vi "Replace Message Specifier.vi"(11 "format string":string) -> (3 "resulting string":string)   [LabVIEW 2018, in "GLog.lvlib" / "Format String.lvclass"]
uses:
  Format String.lvclass
  <vilib>/regexp/Match Regular Expression.xnode
panel:
  # "Connector Pane"
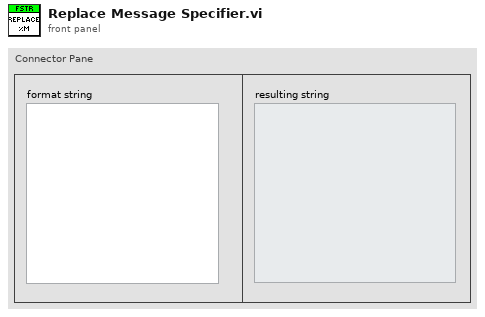
[diagram p1: front panel]
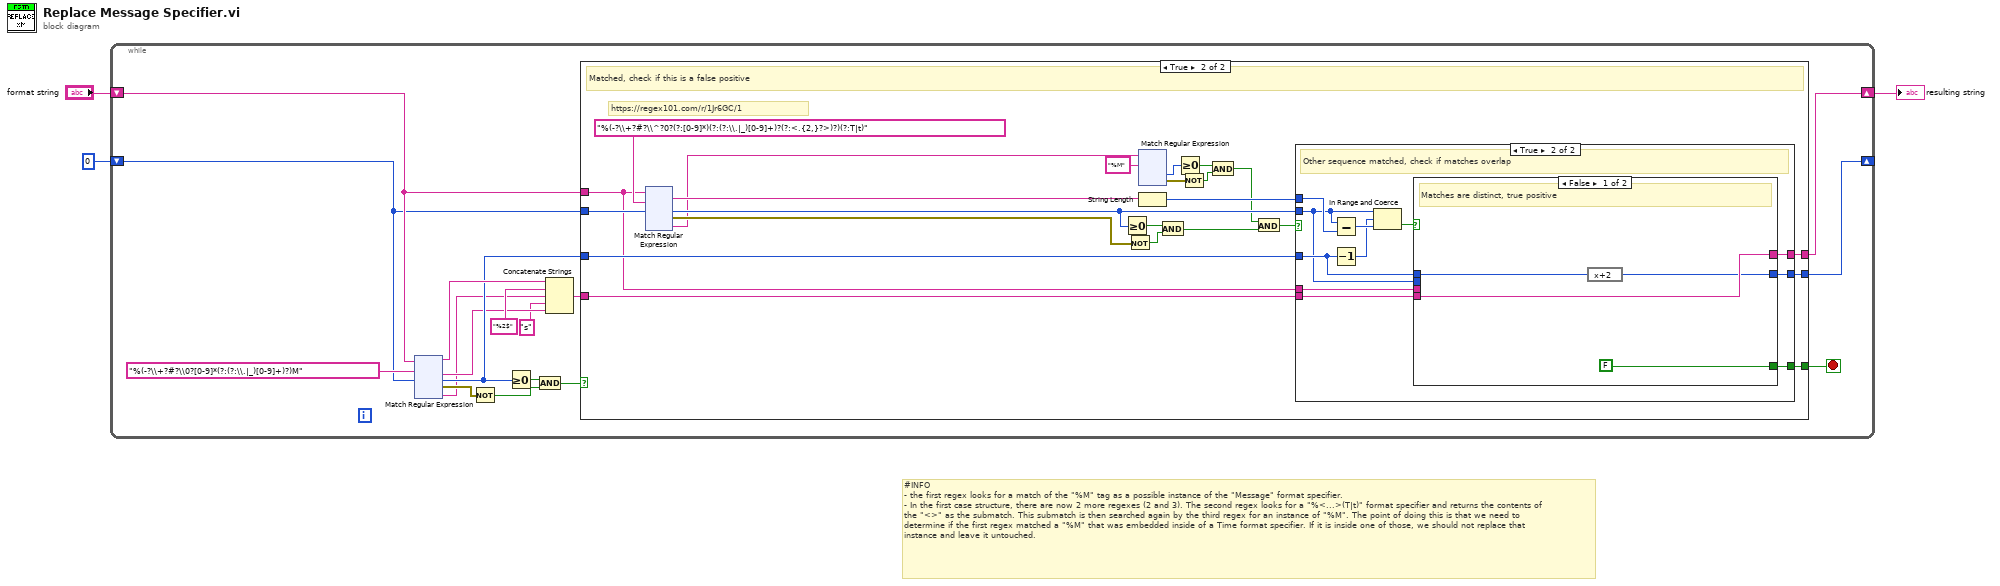
[diagram p0: block diagram]
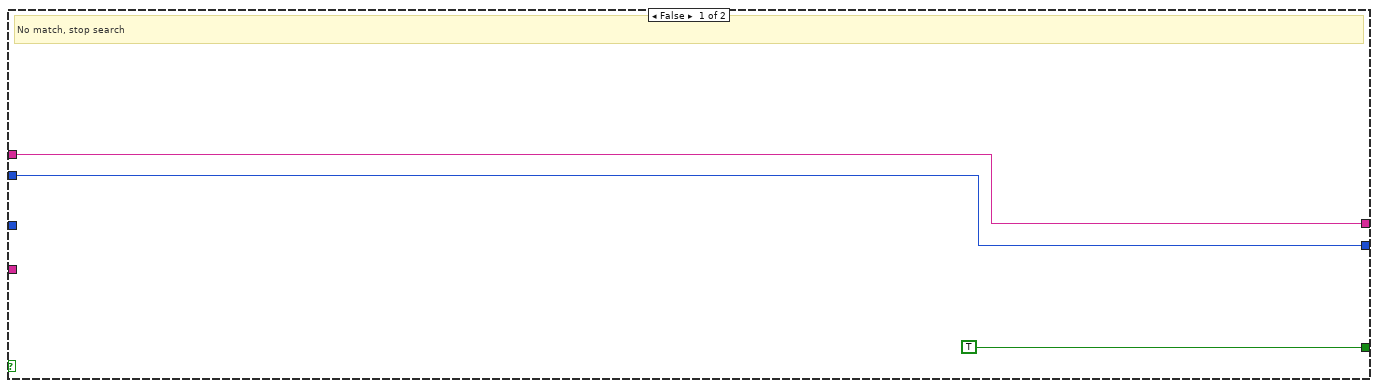
[diagram p2: hidden frame]
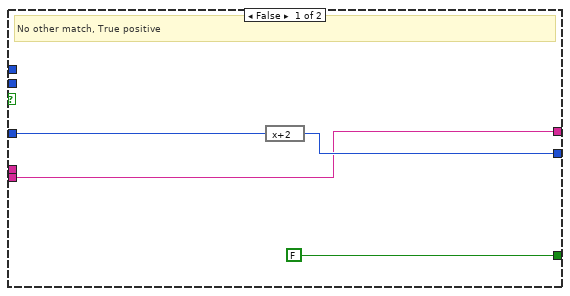
[diagram p3: hidden frame]
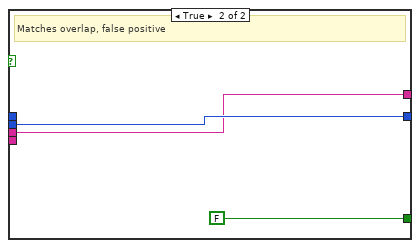
[diagram p4: hidden frame]
diagram:
  # "#INFO\n- the first regex looks for a match of the \"%M\" tag as a possible instance of the \"Message\" format specifier. \n- In the first case structure, there are now 2 more regexes (2 and 3). The second regex looks for a \"%<...>(T|t)\" format specifier and returns the contents of the \"<>\" as the submatch. This submatch is then searched again by the third regex for an instance of \"%M\". The point of doing this is that we need to determine if the first regex matched a \"%M\" that was embedded inside of a Time format specifier. If it is inside one of those, we should not replace that instance and leave it untouched."
  n1 = while {
    shift-right: [w9] -> w2
    shift-left: "format string" -> [w15]
    shift-right: [w8] -> _
    shift-left: 0 ("offset (0)") -> [w14]
    stop <- w10 stop-if-true
    n2 = xnode "Match Regular Expression"("input string"=w15, "regular expression"="%(-?\\+?#?\\0?[0-9]*(?:(?:\\.|_)[0-9]+)?)M", "offset (0)"=w14) -> ("before match"=w16:string, "after match"=w6:string, "offset past match"=w11:i32, "error out"=w18:errorcluster, "submatch 1"=w4:string)  [unwired: 3 in, 1 out]
    n3 = Not(x=w18) -> (.not. x?=w17:bool)
    n4 = Greater Or Equal To 0?(x=w11) -> (x >= 0?=w19:bool)
    n5 = And(x=w19, y=w17) -> (x .and. y?=w12:bool)
    n6 = Concatenate Strings(w16, "%2$" ("string"), w4, "s" ("string"), w6) -> (w7:string)
    n7 = case shown="True" w12 {
      tunnel: w15 -> [w22 w35]
      tunnel: w14 -> [w21 w46]
      tunnel: w11 -> [_ w39]
      tunnel: [TRUE w34] -> w10
      tunnel: [w22 w36] -> w9
      tunnel: [w21 w38] -> w8
      tunnel: w7 -> [_ w37]
      frame False {
        # "No match, stop search"
      }
      frame True {
        # "https://regex101.com/r/1Jr6GC/1"
        # "Matched, check if this is a false positive"
        n8 = xnode "Match Regular Expression"("input string"=w35, "regular expression"="%(-?\\+?#?\\^?0?(?:[0-9]*)(?:(?:\\.|_)[0-9]+)?(?:<.{2,}?>)?)(?:T|t)", "offset (0)"=w46) -> ("whole match"=w33:string, "offset past match"=w41:i32, "error out"=w42:errorcluster, "submatch 1"=w24:string)  [unwired: 3 in, 2 out]
        n9 = Greater Or Equal To 0?(x=w41) -> (x >= 0?=w43:bool)
        n10 = Not(x=w42) -> (.not. x?=w44:bool)
        n11 = xnode "Match Regular Expression"("input string"=w24, "regular expression"="%M") -> ("offset past match"=w29:i32, "error out"=w28:errorcluster)  [unwired: 4 in, 3 out]
        n12 = String Length(string=w33) -> (length=w40:i32)
        n13 = And(x=w43, y=w44) -> (x .and. y?=w26:bool)
        n14 = Greater Or Equal To 0?(x=w29) -> (x >= 0?=w31:bool)
        n15 = Not(x=w28) -> (.not. x?=w30:bool)
        n16 = And(x=w31, y=w30) -> (x .and. y?=w25:bool)
        n17 = And(x=w25, y=w26) -> (x .and. y?=w27:bool)
        n18 = case shown="True" w27 {
          tunnel: w41 -> [_ w289]
          tunnel: w40 -> [_ w297]
          tunnel: w39 -> [w285 w292]
          tunnel: [w286 w293] -> w38
          tunnel: w37 -> [w284 w290]
          tunnel: [w284 w291] -> w36
          tunnel: w35 -> [_ w288]
          tunnel: [FALSE w287] -> w34
          frame False {
            # "No other match, True positive"
            n19 = expression code="x+2"(w285) -> (w286:i32)
          }
          frame True {
            # "Other sequence matched, check if matches overlap"
            n20 = Subtract(x=w289, y=w297) -> (x-y=w296:i32)
            n21 = Decrement(x=w292) -> (x-1=w295:i32)
            n22 = In Range and Coerce(upper limit=w289, x=w295, lower limit=w296) -> (In Range?=w294:bool)  [unwired: 1 out]
            n23 = case shown="False" w294 {
              tunnel: [w299 w304] -> w293
              tunnel: w292 -> [w301 _]
              tunnel: [w300 w303] -> w291
              tunnel: w290 -> [w300 _]
              tunnel: w289 -> [_ w304]
              tunnel: w288 -> [_ w303]
              tunnel: [FALSE FALSE] -> w287
              frame False {
                # "Matches are distinct, true positive"
                n24 = expression code="x+2"(w301) -> (w299:i32)
              }
              frame True {
                # "Matches overlap, false positive"
              }
            }
          }
        }
      }
    }
  }
  "resulting string" <- w2
